vi "Receive Data Loop.vi"(10 "connection ID":refnum<k5>, 11 "队列输入":refnum<queue>) -> ()   [LabVIEW 2020, in "TCP Communication.lvlib"]
uses:
  TCP Communication.lvlib
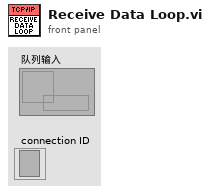
[diagram p1: front panel]
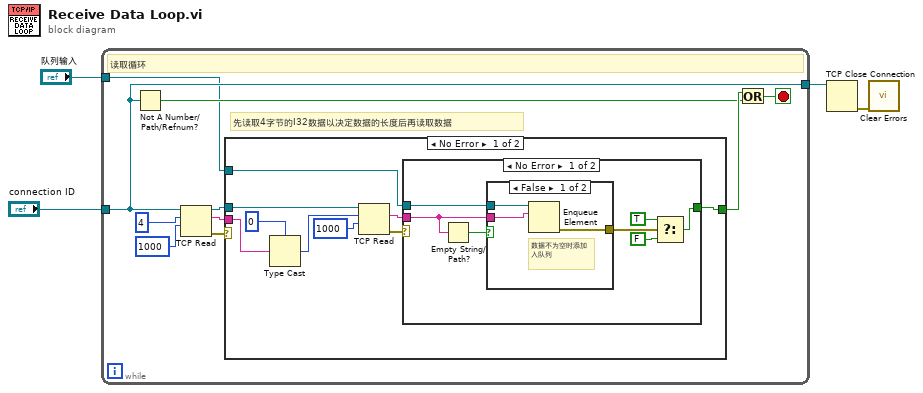
[diagram p0: block diagram]
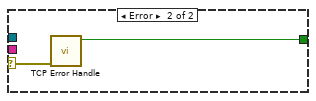
[diagram p3: hidden frame]
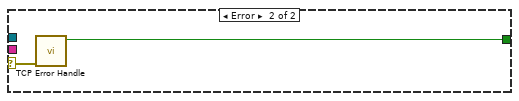
[diagram p4: hidden frame]
diagram:
  n1 = while {
    tunnel: "connection ID" -> [w6]
    tunnel: [w6] -> w1
    tunnel: "队列输入" -> [w5]
    stop <- w9 stop-if-true
    # "先读取4字节的I32数据以决定数据的长度后再读取数据"
    # "读取循环"
    n2 = Not A Number/Path/Refnum?(number/path/refnum=w6) -> (NaN/Path/Refnum?=w7:bool)
    n3 = TCP Read(connection ID=w6, bytes to read=4 ("读取的字节"), 9:1000 ("超时毫秒(25000)")) -> (connection ID out=w10:refnum<k5>, data out=w11:string, error out=w12:errorcluster)  [unwired: 2 in]
    n4 = case shown="No Error" w12 {
      selector: w12 -> [_ w37]
      tunnel: w11 -> [w22 _]
      tunnel: w10 -> [w19 _]
      tunnel: [w15 w36] -> w8
      tunnel: w5 -> [w16 _]
      frame No Error {
        n5 = Type Cast(type=0, x=w22) -> (*(type *) &x=w21:i32)
        n6 = TCP Read(connection ID=w19, bytes to read=w21, 9:1000 ("超时毫秒(25000)")) -> (data out=w17:string, error out=w18:errorcluster)  [unwired: 2 in, 1 out]
        n7 = case shown="No Error" w18 {
          selector: w18 -> [_ w35]
          tunnel: w17 -> [w28 _]
          tunnel: w16 -> [w29 _]
          tunnel: [w26 w34] -> w15
          frame No Error {
            n8 = Empty String/Path?(string/path=w28) -> (empty?=w30:bool)
            n9 = case shown="False" w30 {
              tunnel: w29 -> [w33 _]
              tunnel: w28 -> [w32 _]
              tunnel: [w31 _] -> w27
              frame False {
                # "数据不为空时添加入队列"
                n10 = Enqueue Element(queue=w33, element=w32) -> (error out=w31:errorcluster)  [unwired: 2 in, 2 out]
              }
              frame True {
              }
            }
            n11 = Select(t=TRUE, s=w27, f=FALSE) -> (s? t:f=w26:bool)
          }
          frame Error {
            n12 = call "TCP Error Handle.vi"("错误输入（无错误）"=w35) -> ("Stop?"=w34:bool)  [unwired: 9 in, 1 out]
          }
        }
      }
      frame Error {
        n13 = call "TCP Error Handle.vi"("错误输入（无错误）"=w37) -> ("Stop?"=w36:bool)  [unwired: 9 in, 1 out]
      }
    }
    n14 = Or(x=w8, y=w7) -> (x .or. y?=w9:bool)
  }
  n15 = TCP Close Connection(connection ID=w1) -> (error out=w2:errorcluster)  [unwired: 2 in, 1 out]
  n16 = call <vilib>:"Clear Errors.vi"("error in (no error)"=w2) -> ()  [unwired: 5 in, 2 out]
